vi "BangBang_Calculate_PV.vi"(10 "Measurment":dbl, 11 "BANG_BANG":T1 {"Measurment" format="%13.5p"; "Setpoint" format="%13.5p"; "Tolerance" format="%13.5p"}) -> (1 "ControlOutput":dbl, 3 "out BANG_BANG":T1 {"Measurment" format="%13.5p"; "Setpoint" format="%13.5p"; "Tolerance" format="%13.5p"})   [LabVIEW 2019, in "Trajectory_Library.lvlib"]
doc: "Returns the calculated control output.\n \nAlways ensure that your motor controllers are set to \"coast\" before attempting to control them with a bang-bang controller.\n \nInput:\n - BangBang -- Data cluster\n - measurement -- The most recent measurement of the process variable.\n - setpoint -- The setpoint for the process variable.\n\nOutput\n - outBangBang -- Updated data cluster\n - ControlOutput -- The calculated motor output (0 or 1)."
uses:
  Trajectory_Library.lvlib
  TypeDef/BANG_BANG.ctl
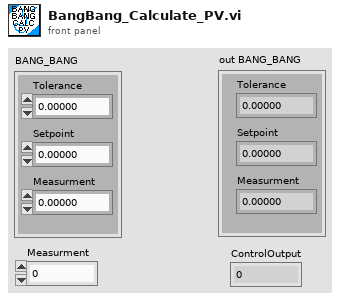
[diagram p1: front panel]
types:
  T1 = typedef "Trajectory_Library.lvlib/BANG_BANG.ctl" = cluster{"Tolerance":dbl, "Setpoint":dbl, "Measurment":dbl}
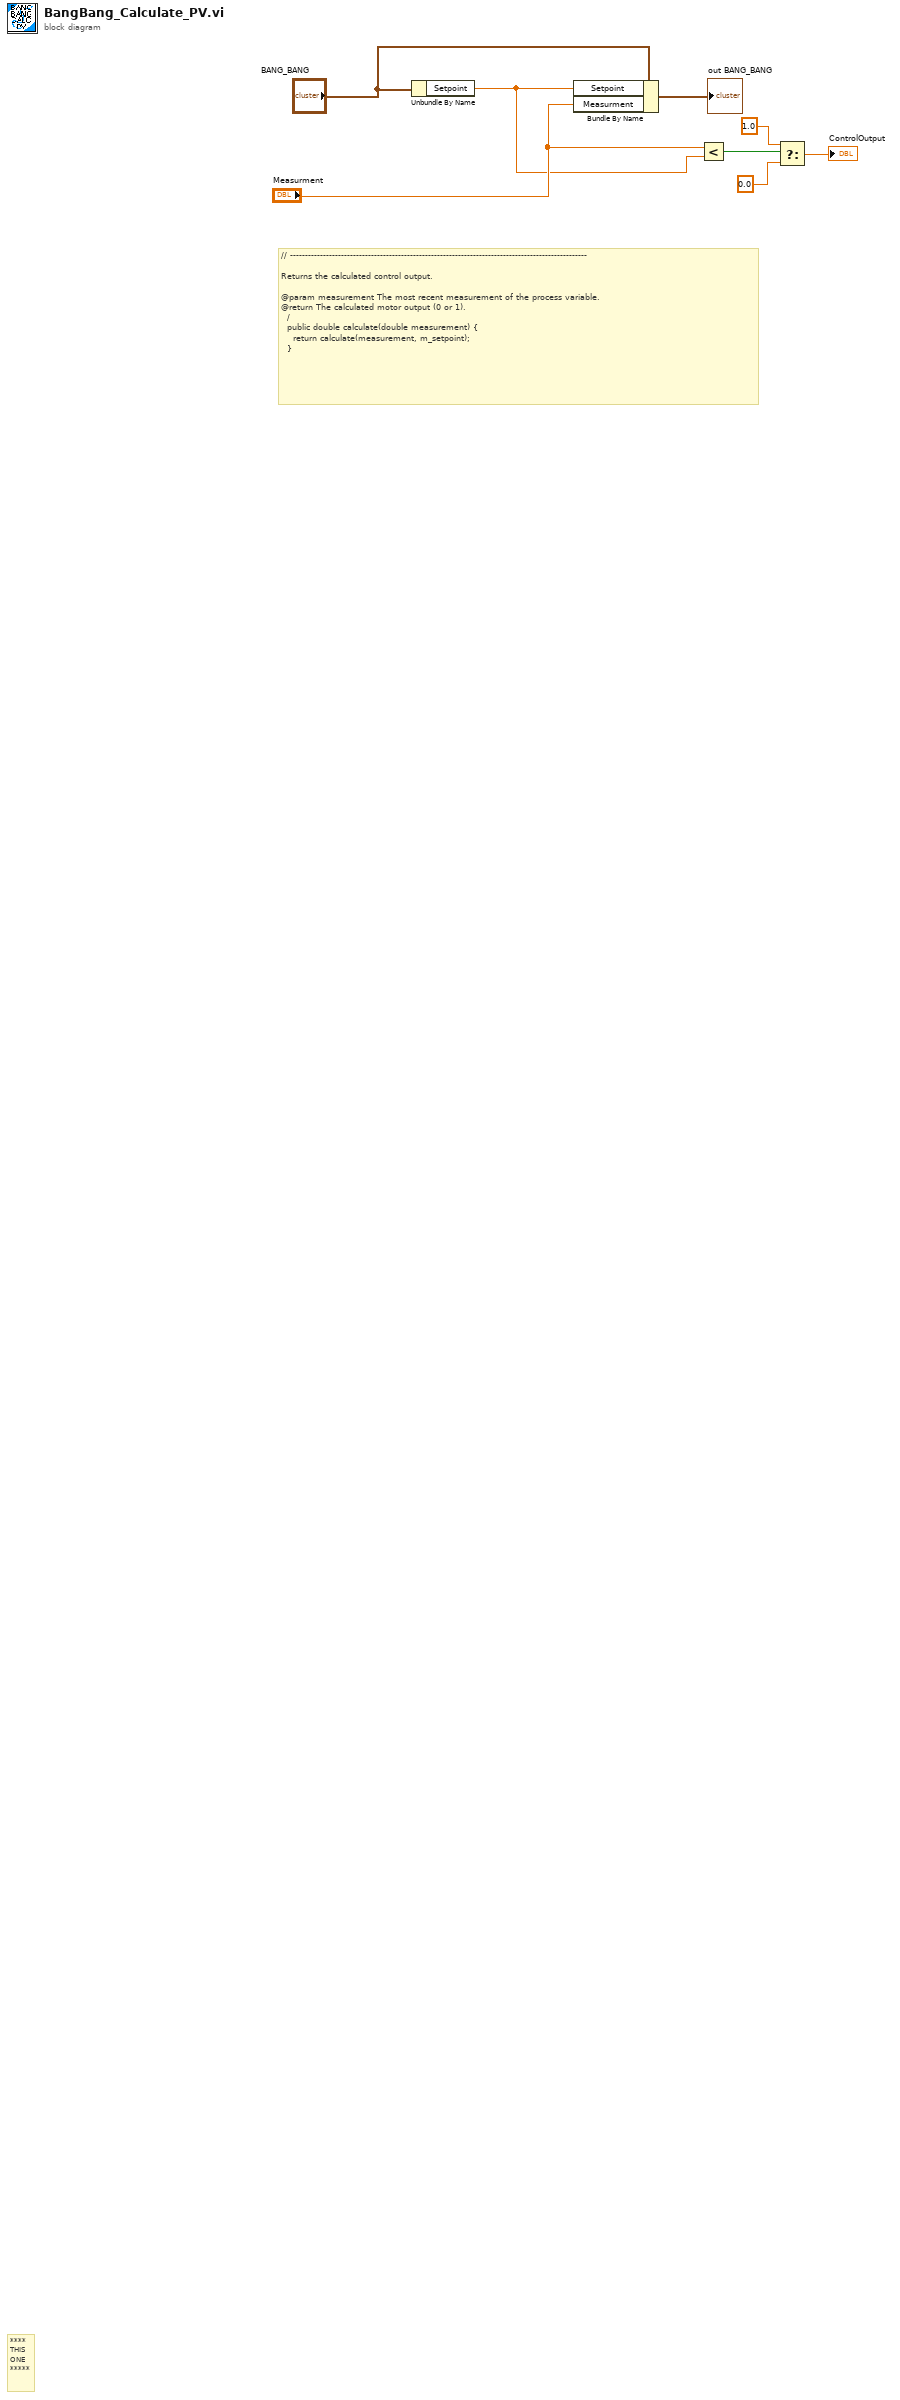
[diagram p0: block diagram]
diagram:
  # "// ---------------------------------------------------------------------------------------------------\n  \nReturns the calculated control output.\n  \n@param measurement The most recent measurement of the process variable.\n@return The calculated motor output (0 or 1).\n  /\n  public double calculate(double measurement) {\n    return calculate(measurement, m_setpoint);\n  }"
  # "****\nTHIS\nONE\n*****"
  n1 = Unbundle By Name("BANG_BANG") -> ("Setpoint"=w1:dbl)
  n2 = Bundle By Name(cluster="BANG_BANG", "Setpoint"=w1, "Measurment"="Measurment") -> (→"out BANG_BANG":T1)
  n3 = Less?(x="Measurment", y=w1) -> (x < y?=w5:bool)
  n4 = Select(t=1.0, s=w5, f=0.0) -> (s? t:f=→"ControlOutput":dbl)
